vi "FX_WriteRaw.vi"(9 "error in (no error)":errorcluster, 10 "Cmd":string, 11 "PLC Conn":refnum<visa-resource-name>) -> (2 "error out":errorcluster, 3 "PLC Conn out":refnum<visa-resource-name>)   [LabVIEW 2018]
doc: "Use this template to build a VI to use as a subVI."
panel:
  # "說明：把佇列字串變成一次寫入。例：D01060004 表示 D106\n 寫 4，後 4 位是十六進位。"
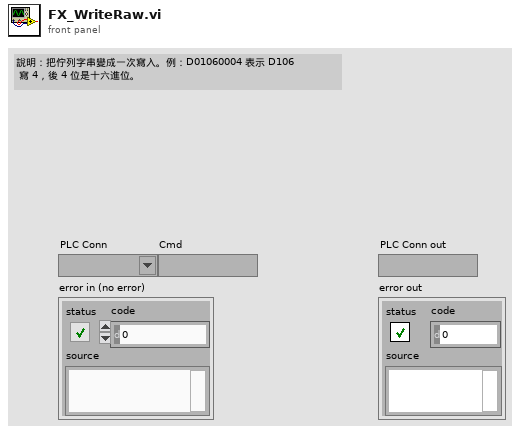
[diagram p1: front panel]
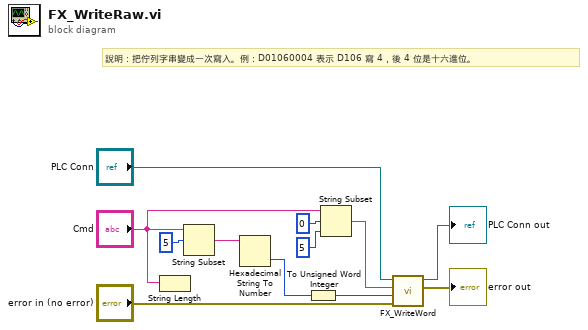
[diagram p0: block diagram]
diagram:
  # "說明：把佇列字串變成一次寫入。例：D01060004 表示 D106 寫 4，後 4 位是十六進位。"
  n1 = String Length(string="Cmd") -> ()  [unwired: 1 out]
  n2 = String Subset(string="Cmd", offset (0)=5) -> (substring=w8:string)  [unwired: 1 in]
  n3 = Hexadecimal String To Number(string=w8) -> (number=w7:u32)  [unwired: 2 in, 1 out]
  n4 = To Unsigned Word Integer(number=w7) -> (unsigned 16bit integer=w5:u16)
  n5 = String Subset(string="Cmd", offset (0)=0, length (rest)=5 ("length (rest)")) -> (substring=w6:string)
  n6 = call "FX_WriteWord.vi"("error in (no error)"="error in (no error)", "Value"=w5, "Device"=w6, "PLC Conn"="PLC Conn") -> ("error out"=→"error out":errorcluster, "PLC Conn out"=→"PLC Conn out":refnum<visa-resource-name>)  [unwired: 6 in]
